vi "loop_with_message_channel.vi"() -> ()   [LabVIEW 2021]
uses:
  <extravilib>/ChannelInstances/Messenger-c(dbl,i32)/Write With Abort.vi
  <extravilib>/ChannelInstances/Messenger-c(dbl,i32)/Read With Abort.vi
  <extravilib>/ChannelInstances/Messenger-c(dbl,i32)/Instantiate.vi
  <extravilib>/ChannelInstances/Messenger-c(dbl,i32)/Endpoint.vi
  <extravilib>/ChannelInstances/Messenger-c(dbl,i32).lvlib
panel:
  out "Waveform Chart":cluster{dbl, dbl}(graph)
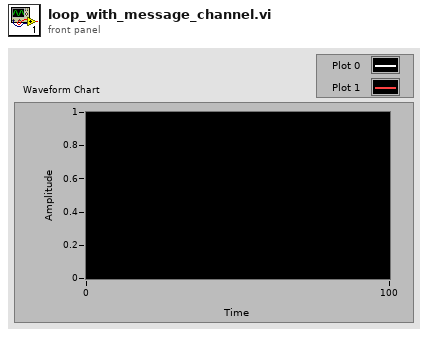
[diagram p1: front panel]
types:
  T1 = typedef "Messenger-c(dbl,i32).lvlib/))Channel.ctl" = refnum<queue>
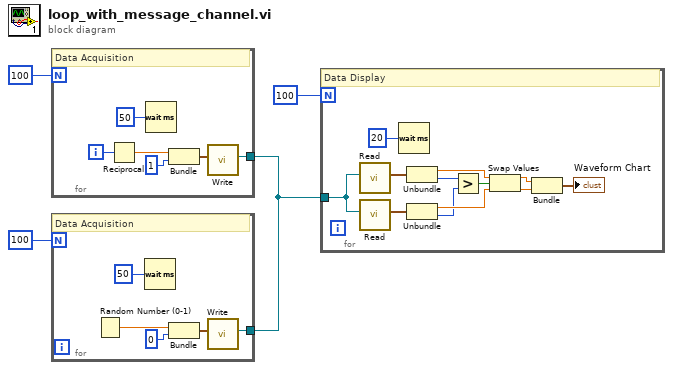
[diagram p0: block diagram]
diagram:
  n1 = for {
    N: 100 -> [_]
    tunnel: [w5] -> w1
    i -> [w9]
    # "Data Acquisition"
    n2 = Reciprocal(x=w9) -> (1/x=w8:dbl)
    n3 = Wait (ms)(milliseconds to wait=u32 50) -> ()  [unwired: 1 out]
    n4 = Bundle(w8, 1) -> (w6:cluster{dbl, i32})  [unwired: 1 in]
    n5 = call <extravilib>:"Write.vi"("element"=w6) -> ("channel"=w5:T1)  [unwired: 8 in, 2 out]
  }
  n6 = for {
    N: 100 -> [_]
    tunnel: w1 -> [w11]
    # "Data Acquisition"
    n7 = Random Number (0-1)() -> (number: 0 to 1=w14:dbl)
    n8 = Wait (ms)(milliseconds to wait=u32 50) -> ()  [unwired: 1 out]
    n9 = Bundle("number: 0 to 1"=w14, 0) -> (w12:cluster{"number: 0 to 1":dbl, i32})  [unwired: 1 in]
    n10 = call <extravilib>:"Write.vi"("element"=w12) -> ("channel"=w11:T1)  [unwired: 8 in, 2 out]
  }
  n11 = for {
    N: 100 -> [_]
    tunnel: w1 -> [w26]
    # "Data Display"
    n12 = call <extravilib>:"Read.vi"("channel"=w26) -> ("element"=w25:cluster{"number: 0 to 1":dbl, i32})  [unwired: 8 in, 2 out]
    n13 = call <extravilib>:"Read.vi"("channel"=w26) -> ("element"=w24:cluster{"number: 0 to 1":dbl, i32})  [unwired: 8 in, 2 out]
    n14 = Wait (ms)(milliseconds to wait=u32 20) -> ()  [unwired: 1 out]
    n15 = Unbundle(w25) -> ("number: 0 to 1"=w23:dbl, w21:i32)
    n16 = Unbundle(w24) -> ("number: 0 to 1"=w22:dbl, w20:i32)
    n17 = Greater?(x=w21, y=w20) -> (0:w19:bool)
    n18 = Swap Values(12:w23, 13:w19, 14:w22) -> (1:w18:dbl, 3:w17:dbl)
    n19 = Bundle(w18, w17) -> (→"Waveform Chart":cluster{dbl, dbl})  [unwired: 1 in]
  }
